vi "DAQ.measureInputOffset.vi"(8 "error in (no error)":errorcluster, 10 "measureInputOffset":T1={"buffers"=10, "settle"=2, "timeout"=5.0, "channels"=[], "zero"=enum."both"}, 11 "Instrument.DAQ":refnum<class "Instrument.DAQ.lvclass">) -> (0 "error out":errorcluster, 3 "Instrument.DAQ out":refnum<class "Instrument.DAQ.lvclass">)   [LabVIEW 2019, in "Instrument.Lockin.lvlib" / "Instrument.DAQ.lvclass"]
doc: "---------------------------------------------------------------\nJKI State Machine Objects™\nhttp://jki.net/state-machine-objects/\nCopyright (C) 2005-2015, JKI <info@jki.net>\nALL RIGHTS RESERVEDJKI State Machine Objects (SMO) 1.0.0.4\nJKI - JKI\nCopyright (c) 2015, JKI"
uses:
  Instrument.DAQ.lvclass
  Lockin.Typedefs/API/Lockin.measureInputOffset Config--Cluster.ctl
  Lockin.Typedefs/API/Lockin.measureInputOffset.zero--enum.ctl
  Typedefs/PrivateEvents--DAQ.measureInputOffset.ctl
  Instrument.DAQ.lvclass/Instrument.DAQ.ctl
  Lockin.Typedefs/Lockin.Typedefs.lvlib
panel:
  # "For instructions on how to use the JKI State Machine Objects, examples and video tutorials, visit:\nhttp://jki.net/state-machine-objects/\n\nJKI State Machine Objects™\nhttp://jki.net/state-machine-objects/\nCopyright (C) 2005-2015, JKI <info@jki.net>\nALL RIGHTS RESERVED"
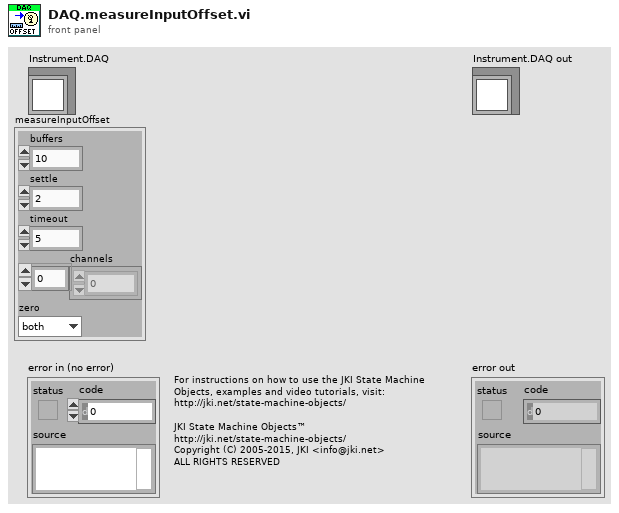
[diagram p1: front panel]
types:
  T1 = typedef "Lockin.Typedefs.lvlib/Lockin.measureInputOffset Config--Cluster.ctl" = cluster{"buffers":i32, "settle":i32, "timeout":dbl, "channels":i32[], "zero":T2}
  T2 = typedef "Lockin.Typedefs.lvlib/Lockin.measureInputOffset.zero--enum.ctl" = enum16{"both", "ac", "dc", "none"}
  T3 = typedef "Instrument.Lockin.lvlib/Instrument.DAQ.lvclass/PrivateEvents--DAQ.measureInputOffset.ctl" = cluster{"measureInputOffset":T1}
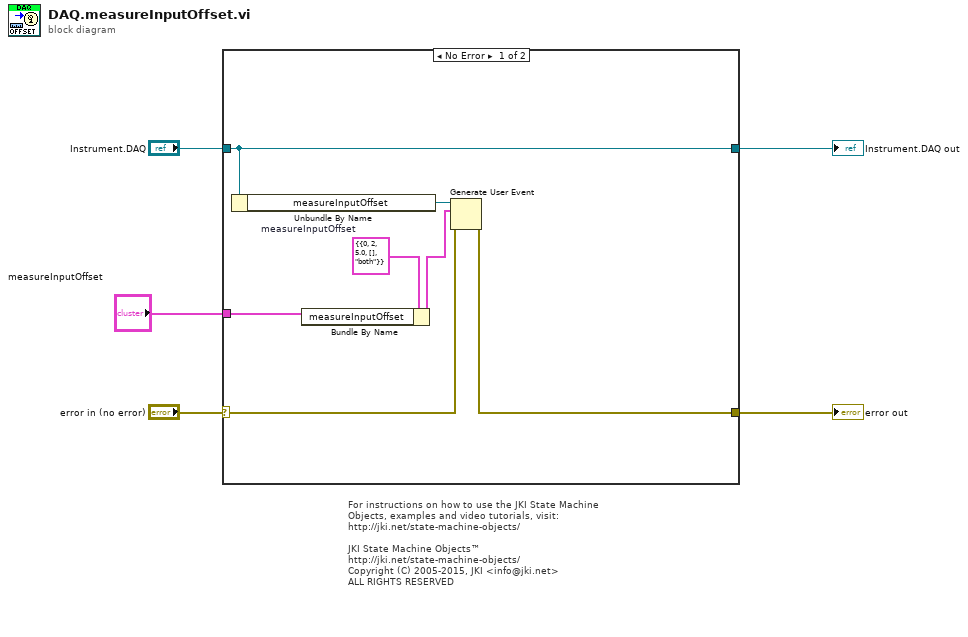
[diagram p0: block diagram]
diagram:
  # "For instructions on how to use the JKI State Machine Objects, examples and video tutorials, visit:\nhttp://jki.net/state-machine-objects/\n\nJKI State Machine Objects™\nhttp://jki.net/state-machine-objects/\nCopyright (C) 2005-2015, JKI <info@jki.net>\nALL RIGHTS RESERVED"
  n1 = case shown="No Error" "error in (no error)" {
    selector: "error in (no error)" -> [w12 w14]
    tunnel: [w10 w14] -> w4
    tunnel: [w9 w13] -> w5
    tunnel: "Instrument.DAQ" -> [w9 w13]
    tunnel: "measureInputOffset" -> [w6 _]
    frame No Error {
      w8 = T3 {"measureInputOffset"={"buffers"=0, "settle"=2, "timeout"=5.0, "channels"=[], "zero"=enum."both"}}  # measureInputOffset
      n2 = Unbundle By Name(w9) -> ("measureInputOffset"=w11:refnum<user-event>)
      n3 = Bundle By Name(cluster=w8, "measureInputOffset"=w6) -> (w7:T3)
      n4 = Generate User Event(user event=w11, event data cluster=w7, error in=w12) -> (error out=w10:errorcluster)  [unwired: 1 in, 1 out]
    }
    frame Error {
    }
  }
  "error out" <- w4
  "Instrument.DAQ out" <- w5
